vi "Create Group.vi"(5 "Save File":bool=TRUE, 6 "error in (no error)":errorcluster, 8 "Group Name":string, 9 "EasyUserManager in":refnum<class "EasyUserManager.lvclass">) -> (0 "error out":errorcluster, 3 "EasyUserManager out":refnum<class "EasyUserManager.lvclass">)   [LabVIEW 2024, in "EasyUserManager.lvclass"]
doc: "Create a new Teststand Group with the provided <B>Group Name</B>. The group is added to the user group list of the current users file. \n\nThe boolean input <B>Save File</B> controls whether changes are immediately saved to the users file (Default: True)."
uses:
  EasyUserManager.lvclass
  EasyUserManager.lvclass/EasyUserManager.ctl
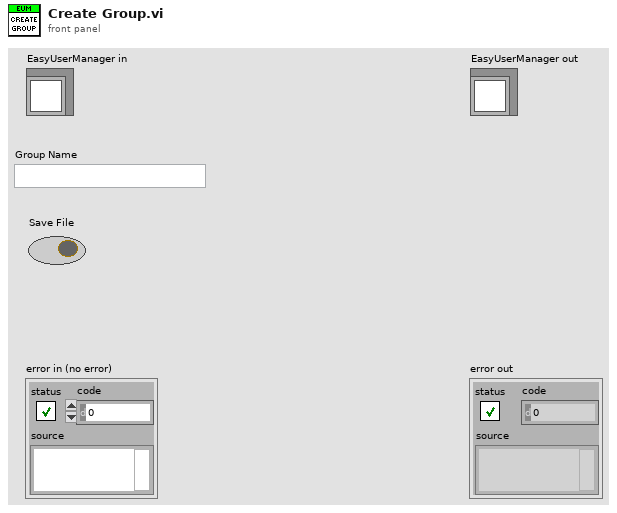
[diagram p1: front panel]
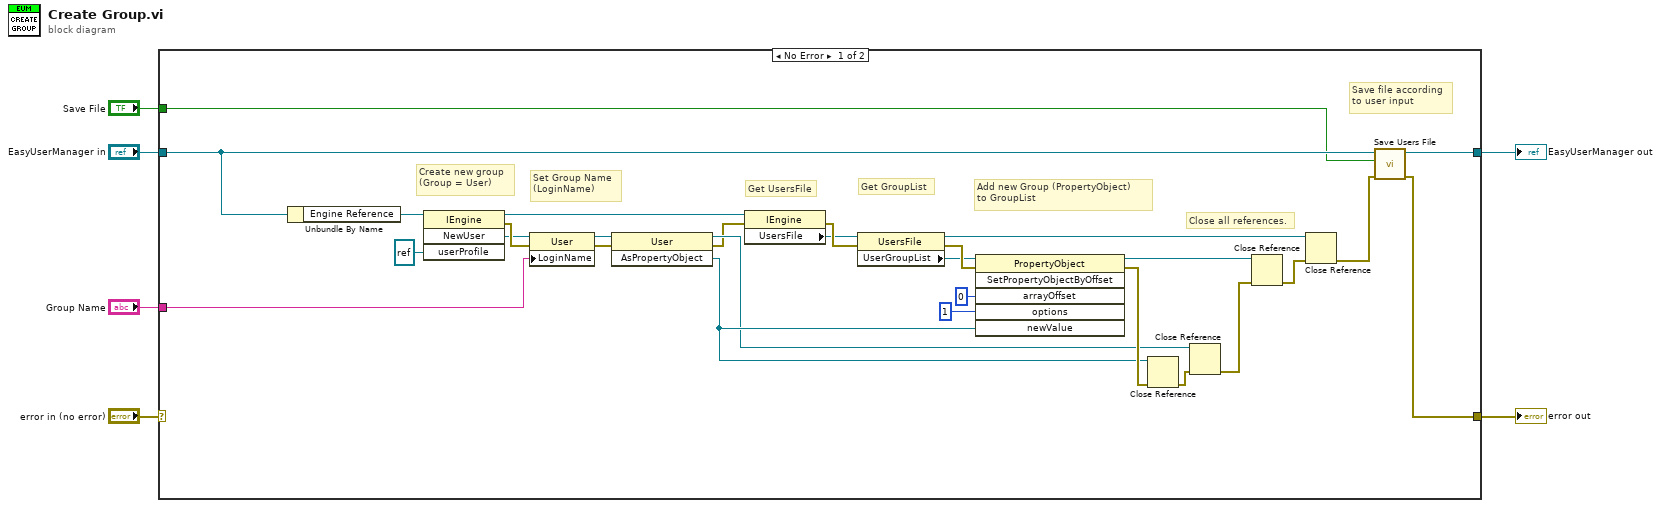
[diagram p0: block diagram]
diagram:
  n1 = case shown="No Error" "error in (no error)" {
    selector: "error in (no error)" -> [_ w36]
    tunnel: [w9 w36] -> w5
    tunnel: [w12 w35] -> w3
    tunnel: "EasyUserManager in" -> [w11 w35]
    tunnel: "Group Name" -> [w8 _]
    tunnel: "Save File" -> [w7 _]
    frame No Error {
      # "Save file according\nto user input"
      # "Close all references."
      # "Add new Group (PropertyObject)\nto GroupList"
      # "Get GroupList"
      # "Get UsersFile"
      # "Set Group Name\n(LoginName)"
      # "Create new group\n(Group = User)"
      n2 = Unbundle By Name(w11) -> ("Engine Reference"=w13:refnum<k7>)
      n3 = invoke on="Invoke Node" class="IEngine" method="NewUser"(reference=w13, "userProfile"=refnum<k7> refnum) -> (reference out=w19:refnum<k7>, error out=w18:errorcluster, "NewUser"=w17:refnum<k7>)  [unwired: 2 in, 1 out]
      n4 = property on="Property Node" class="User"(reference=w17, error in=w18, "LoginName"=w8) -> (reference out=w22:refnum<k7>, error out=w23:errorcluster)
      n5 = invoke on="Invoke Node" class="User" method="AsPropertyObject"(reference=w22, error in=w23) -> (reference out=w27:refnum<k7>, error out=w24:errorcluster, "AsPropertyObject"=w28:refnum<k7>)  [unwired: 1 in]
      n6 = property on="Property Node" class="IEngine"(reference=w19, error in=w24) -> (error out=w25:errorcluster, "UsersFile"=w20:refnum<k7>)  [unwired: 1 out]
      n7 = property on="Property Node" class="UsersFile"(reference=w20, error in=w25) -> (reference out=w34:refnum<k7>, error out=w26:errorcluster, "UserGroupList"=w21:refnum<k7>)
      n8 = invoke on="Invoke Node" class="PropertyObject" method="SetPropertyObjectByOffset"(reference=w21, error in=w26, "arrayOffset"=0, "options"=1, "newValue"=w28) -> (reference out=w32:refnum<k7>, error out=w29:errorcluster)  [unwired: 1 in, 4 out]
      n9 = Close Reference(reference=w28, error in (no error)=w29) -> (error out=w30:errorcluster)
      n10 = Close Reference(reference=w27, error in (no error)=w30) -> (error out=w31:errorcluster)
      n11 = Close Reference(reference=w32, error in (no error)=w31) -> (error out=w33:errorcluster)
      n12 = Close Reference(reference=w34, error in (no error)=w33) -> (error out=w10:errorcluster)
      n13 = call "Save Users File.vi"("error in (no error)"=w10, "Save"=w7, "EasyUserManager in"=w11) -> ("error out"=w9:errorcluster, "EasyUserManager out"=w12:refnum<class "EasyUserManager.lvclass">)  [unwired: 3 in]
    }
    frame Error {
      # "Pass error and do nothing."
    }
  }
  "error out" <- w5
  "EasyUserManager out" <- w3
